vi "detect modules.vi"(8 "error in":errorcluster, 10 "C Series module in":refnum<class "C Series Module.lvclass">, 11 "chassis in":refnum<class "Chassis.lvclass">) -> (0 "error out":errorcluster, 2 "C Series module out":refnum<class "C Series Module.lvclass">, 3 "chassis out":refnum<class "Chassis.lvclass">)   [LabVIEW 2014, in "SMI.lvlib" / "C Series Module.lvclass"]
uses:
  C Series Module.lvclass
  Chassis/Chassis.lvclass
  <vilib>/FPGAPlugInAG/Dynamic/niLvFpga_Close_Dynamic.vi
  <vilib>/FPGAPlugInAG/Dynamic/niLvFpga_Run_Dynamic.vi
  <vilib>/FPGAPlugInAG/Dynamic/niLvFpga_Reset_Dynamic.vi
  Device/read device class.vi
  Device/read product name.vi
  <vilib>/regexp/Match Regular Expression.xnode
  <vilib>/rvi/interface/nirviCloseFPGA/nirviCloseFPGA.xnode
  <vilib>/rvi/interface/nirviMethod/nirviMethod.xnode
  Module/Module.lvclass
  SMI.lvlib
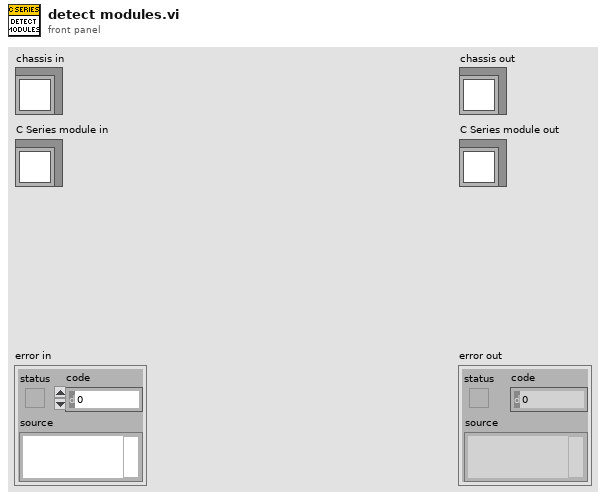
[diagram p1: front panel]
types:
  T1 = typedef "SMI.lvlib/Module.lvclass/module information.ctl" = cluster{"vendor name":string, "product name":string, "product ID":u16, "serial number":string}
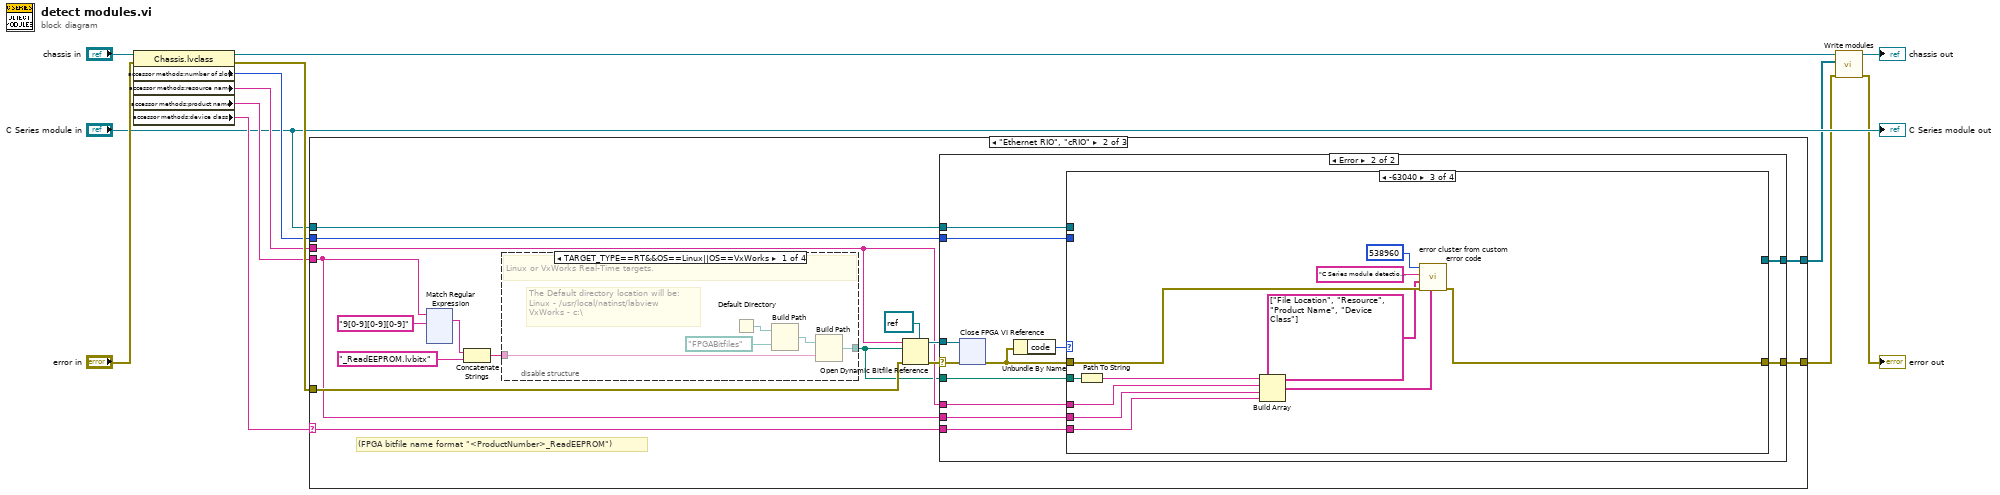
[diagram p0: block diagram]
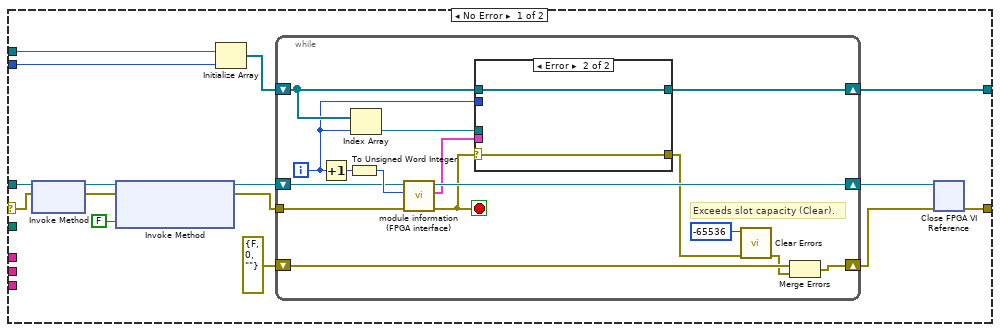
[diagram p3: hidden frame]
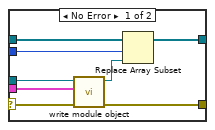
[diagram p4: hidden frame]
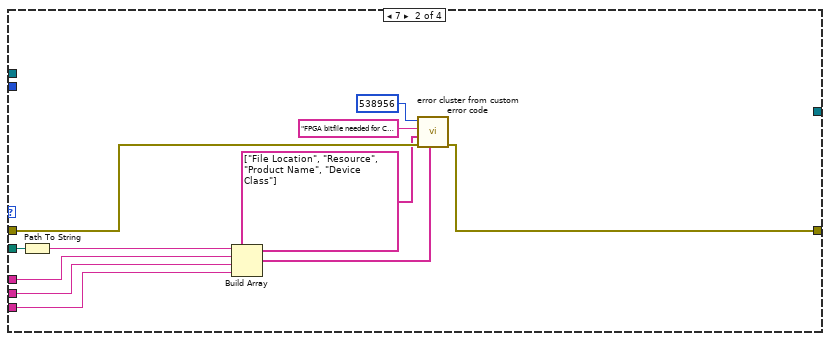
[diagram p6: hidden frame]
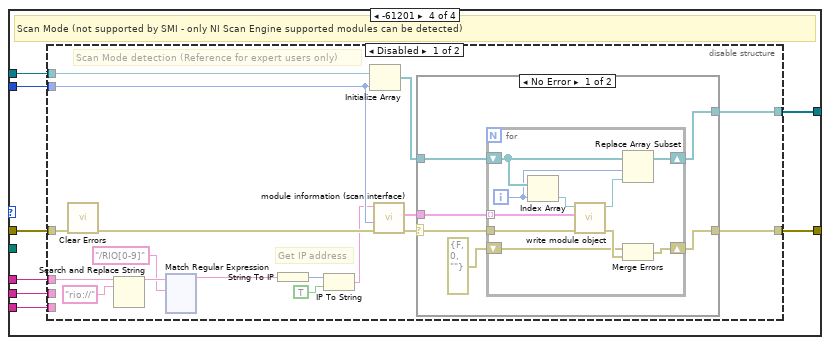
[diagram p7: hidden frame]
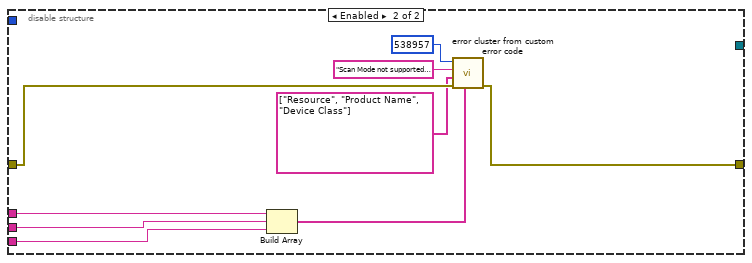
[diagram p9: hidden frame]
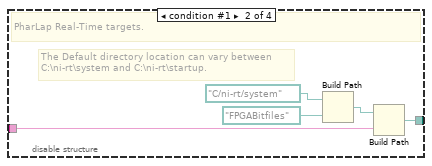
[diagram p10: hidden frame]
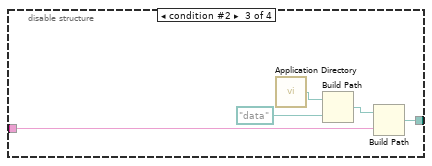
[diagram p11: hidden frame]
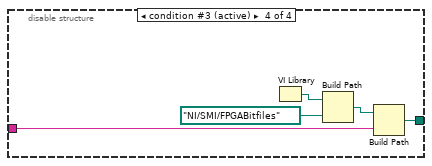
[diagram p12: hidden frame]
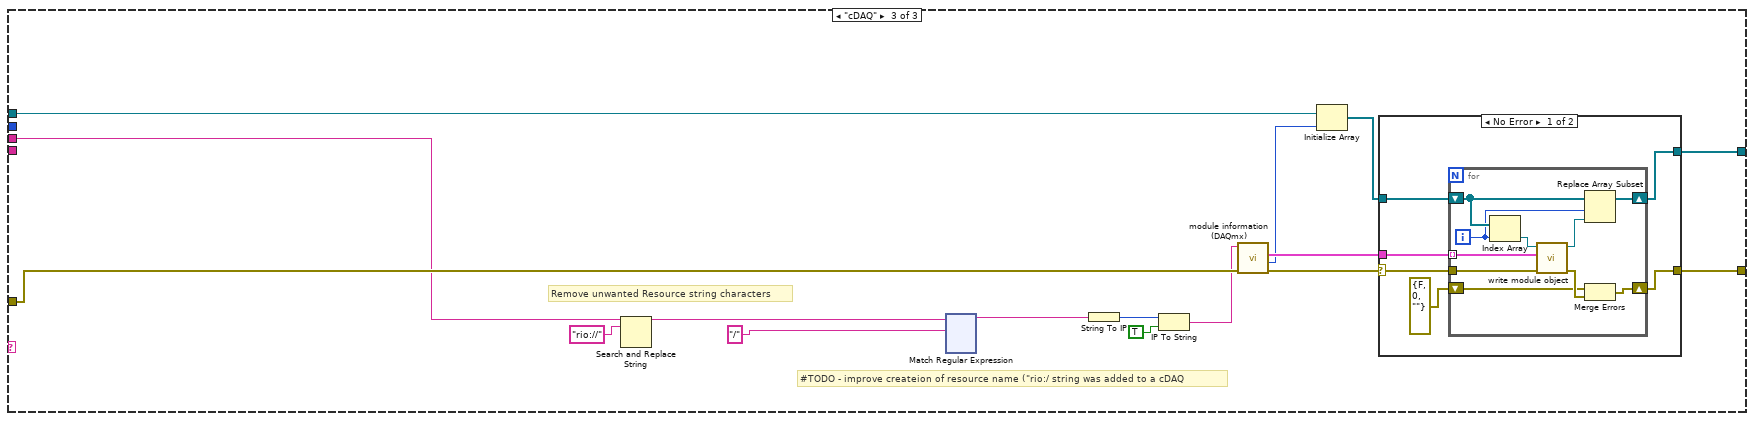
[diagram p13: hidden frame]
diagram:
  n1 = property class="Chassis.lvclass"(reference="chassis in", error in="error in") -> (reference out=w6:refnum<class "Chassis.lvclass">, error out=w12:errorcluster, "accessor methods:number of slots"=w7:i32, "accessor methods:resource name"=w8:string, "accessor methods:product name"=w9:string, "accessor methods:device class"=w10:string)
  n2 = case shown="\"Ethernet RIO\", \"cRIO\"" w10 {
    selector: w10 -> [_ w15 _]
    tunnel: [w14 w19 w418] -> w2
    tunnel: w12 -> [w14 w26 w421]
    tunnel: w9 -> [_ w16 _]
    tunnel: w8 -> [_ w18 w417]
    tunnel: w7 -> [_ w22 _]
    tunnel: "C Series module in" -> [_ w23 w420]
    tunnel: [_ w20 w419] -> w3
    frame Default {
      # "#TODO - Re-create block diagram (from lv2016 reference)."
    }
    frame "Ethernet RIO", "cRIO" {
      # "(FPGA bitfile name format \"<ProductNumber>_ReadEEPROM\")"
      n3 = xnode "Match Regular Expression"("input string"=w16, "regular expression"="9[0-9][0-9][0-9]") -> ("whole match"=w29:string)  [unwired: 4 in, 4 out]
      n4 = Concatenate Strings(w29, "_ReadEEPROM.lvbitx" ("string")) -> (w27:string)
      n5 = disable-structure shown="TARGET_TYPE==RT&&OS==Linux||OS==VxWorks" {
        disable-tunnel: w27 -> [w273 w279 w284 w288]
        disable-tunnel: [w272 w278 w283 w287] -> w17
        frame condition #0 {
          # "The Default directory location will be:\nLinux - /usr/local/natinst/labview\nVxWorks - c:\\"
          # "Linux or VxWorks Real-Time targets."
          n6 = Default Directory() -> (w276:path)
          n7 = Build Path(base path=w276, name or relative path=path "FPGABitfiles") -> (appended path=w274:path)
          n8 = Build Path(base path=w274, name or relative path=w273) -> (appended path=w272:path)
        }
        frame condition #1 {
          # "The Default directory location can vary between\nC:\\ni-rt\\system and C:\\ni-rt\\startup."
          # "PharLap Real-Time targets."
          n9 = Build Path(base path=path "C:/ni-rt/system", name or relative path=path "FPGABitfiles") -> (appended path=w280:path)
          n10 = Build Path(base path=w280, name or relative path=w279) -> (appended path=w278:path)
        }
        frame condition #2 {
          n11 = call <vilib>:"Application Directory.vi"() -> ("Application Directory"=w282:path)
          n12 = Build Path(base path=w282, name or relative path=path "data") -> (appended path=w285:path)
          n13 = Build Path(base path=w285, name or relative path=w284) -> (appended path=w283:path)
        }
        frame condition #3 (active) {
          n14 = VI Library() -> (path=w291:path)
          n15 = Build Path(base path=w291, name or relative path=path "NI/SMI/FPGABitfiles") -> (appended path=w289:path)
          n16 = Build Path(base path=w289, name or relative path=w288) -> (appended path=w287:path)
        }
      }
      n17 = Open Dynamic Bitfile Reference(0:w18, 1:w17, 3:w26, 4:refnum<k20> refnum ("Refnum in")) -> (5:w24:refnum<k20>, 8:w25:errorcluster)  [unwired: 1 in]
      n18 = case shown="Error" w25 {
        selector: w25 -> [w36 w75]
        tunnel: w24 -> [w37 w76]
        tunnel: w23 -> [w45 w82]
        tunnel: w22 -> [w44 w81]
        tunnel: [w42 w79] -> w20
        tunnel: [w38 w78] -> w19
        tunnel: w18 -> [_ w80]
        tunnel: w17 -> [_ w77]
        tunnel: w16 -> [_ w72]
        tunnel: w15 -> [_ w73]
        frame No Error {
          n19 = xnode "Invoke Method"("FPGA VI Reference In"=w37, "error in"=w36) -> ("FPGA VI Reference Out"=w35:refnum<k20>, "error out"=w34:errorcluster)
          n20 = xnode "Invoke Method"("FPGA VI Reference In"=w35, "error in"=w34, "Wait Until Done (F)"=FALSE) -> ("FPGA VI Reference Out"=w33:refnum<k20>, "error out"=w32:errorcluster)
          n21 = Initialize Array(w45, w44) -> (w43:refnum<class "C Series Module.lvclass">[])
          n22 = while {
            shift-right: [w53] -> w42
            shift-left: w43 -> [w54]
            tunnel: w32 -> [w61]
            shift-right: [w57] -> w40
            shift-left: w33 -> [w58]
            shift-right: [w48] -> w39
            shift-left: errorcluster {"status"=FALSE, "code"=0, "source"=""} ("error constant") -> [w49]
            i -> [w52]
            stop <- w51 stop-if-true
            # "Exceeds slot capacity (Clear)."
            n23 = Increment(x=w52) -> (x+1=w60:i32)
            n24 = To Unsigned Word Integer(number=w60) -> (unsigned 16bit integer=w59:u16)
            n25 = Index Array(array=w54, index=w52) -> (element=w56:refnum<class "C Series Module.lvclass">)
            n26 = call "module information (FPGA interface).vi"("error in"=w61, "Module"=w59, "Refnum in"=w58) -> ("error out"=w51:errorcluster, "Module Information"=w55:T1, "Refnum out"=w57:refnum<k20>)  [unwired: 6 in]
            n27 = case shown="Error" w51 {
              selector: w51 -> [w68 w70]
              tunnel: w56 -> [w69 _]
              tunnel: w55 -> [w67 _]
              tunnel: w54 -> [w66 w71]
              tunnel: [w65 w71] -> w53
              tunnel: w52 -> [w63 _]
              tunnel: [w62 w70] -> w50
              frame No Error {
                n28 = call "write module object.vi"("error in"=w68, "module information"=w67, "Module in"=w69) -> ("error out"=w62:errorcluster, "Module out"=w64:refnum<class "C Series Module.lvclass">)  [unwired: 7 in]
                n29 = Replace Array Subset(array=w66, new element=w64, index=w63) -> (w65:refnum<class "C Series Module.lvclass">[])
              }
              frame Error {
              }
            }
            n30 = call <vilib>:"Clear Errors.vi"("error in (no error)"=w50, "specific error code to clear (0: all)"=-65536) -> ("error out"=w47:errorcluster)  [unwired: 4 in, 1 out]
            n31 = Merge Errors(w49, w47) -> (w48:errorcluster)
          }
          n32 = xnode "Close FPGA VI Reference"("FPGA VI Reference In"=w40, "error in"=w39) -> ("error out"=w38:errorcluster)
        }
        frame Error {
          n33 = xnode "Close FPGA VI Reference"("FPGA VI Reference In"=w76, "error in"=w75) -> ("error out"=w74:errorcluster)
          n34 = Unbundle By Name(w74) -> ("code"=w83:i32)
          n35 = case shown="-63040" w83 {
            tunnel: w74 -> [w84 w92 w103 w114]
            tunnel: w82 -> [_ _ _ w113]
            tunnel: w81 -> [_ _ _ w112]
            tunnel: w80 -> [_ w91 w102 w111]
            tunnel: [_ _ _ w110] -> w79
            tunnel: [w84 w94 w105 w109] -> w78
            tunnel: w77 -> [_ w95 w106 _]
            tunnel: w73 -> [_ w89 w100 w107]
            tunnel: w72 -> [_ w90 w101 w108]
            frame Default {
            }
            frame 7 {
              n36 = Path To String(path=w95) -> (string=w93:string)
              n37 = Build Array(w93, w91, w90, w89) -> (w87:string[])
              n38 = call "error cluster from custom error code.vi"("string values"=w87, "error in"=w92, "keys"=string[] ["File Location", "Resource", "Product Name", "Device Class"], "error message"="FPGA bitfile needed for C Series module detection was not found in the expected file location.", "custom error code (0)"=538956 ("error code (0)")) -> ("error out"=w94:errorcluster)  [unwired: 6 in]
            }
            frame -63040 {
              n39 = Path To String(path=w106) -> (string=w104:string)
              n40 = Build Array(w104, w102, w101, w100) -> (w98:string[])
              n41 = call "error cluster from custom error code.vi"("string values"=w98, "error in"=w103, "keys"=string[] ["File Location", "Resource", "Product Name", "Device Class"], "error message"="C Series module detection is not supported for remote chassis connected to a secondary network adapter.", "custom error code (0)"=538960 ("error code (0)")) -> ("error out"=w105:errorcluster)  [unwired: 6 in]
            }
            frame -61201 {
              # "Scan Mode (not supported by SMI - only NI Scan Engine supported modules can be detected)"
              n42 = disable-structure shown="Disabled" {
                disable-tunnel: w114 -> [w131 w268]
                disable-tunnel: w113 -> [w130 _]
                disable-tunnel: w112 -> [w129 _]
                disable-tunnel: w111 -> [w125 w271]
                disable-tunnel: [w120 _] -> w110
                disable-tunnel: [w119 w267] -> w109
                disable-tunnel: w108 -> [_ w270]
                disable-tunnel: w107 -> [_ w269]
                frame Disabled {
                  # "Get IP address"
                  # "Scan Mode detection (Reference for expert users only)"
                  n43 = call <vilib>:"Clear Errors.vi"("error in (no error)"=w131) -> ("error out"=w126:errorcluster)  [unwired: 5 in, 1 out]
                  n44 = Search and Replace String(input string=w125, search string="rio://") -> (result string=w123:string)  [unwired: 6 in, 3 out]
                  n45 = xnode "Match Regular Expression"("input string"=w123, "regular expression"="/RIO[0-9]") -> ("before match"=w116:string)  [unwired: 4 in, 4 out]
                  n46 = String To IP(1:w116) -> (0:w118:u32)
                  n47 = IP To String(1:TRUE ("dot notation? (F)"), 2:w118) -> (0:w115:string)
                  n48 = Initialize Array(w130, w129) -> (w121:refnum<class "C Series Module.lvclass">[])
                  n49 = call "module information (scan interface).vi"("error in"=w126, "number of slots"=w129, "IP address (localhost)"=w115) -> ("error out"=w128:errorcluster, "module information"=w127:T1[])  [unwired: 7 in]
                  n50 = case shown="No Error" w128 {
                    selector: w128 -> [w248 w262]
                    tunnel: w127 -> [w251 _]
                    tunnel: w121 -> [w250 _]
                    tunnel: [w247 _] -> w120
                    tunnel: [w246 w262] -> w119
                    frame No Error {
                      n51 = for {
                        tunnel: w251 -> [w261] mode=indexing
                        shift-right: [w254] -> w247
                        shift-left: w250 -> [w255]
                        shift-right: [w256] -> w246
                        shift-left: errorcluster {"status"=FALSE, "code"=0, "source"=""} ("error constant") -> [w258]
                        tunnel: w248 -> [w260]
                        i -> [w253]
                        n52 = Index Array(array=w255, index=w253) -> (element=w257:refnum<class "C Series Module.lvclass">)
                        n53 = call "write module object.vi"("error in"=w260, "module information"=w261, "Module in"=w257) -> ("error out"=w259:errorcluster, "Module out"=w252:refnum<class "C Series Module.lvclass">)  [unwired: 7 in]
                        n54 = Replace Array Subset(array=w255, new element=w252, index=w253) -> (w254:refnum<class "C Series Module.lvclass">[])
                        n55 = Merge Errors(w258, w259) -> (w256:errorcluster)
                      }
                    }
                    frame Error {
                    }
                  }
                }
                frame Enabled {
                  n56 = Build Array(w271, w270, w269) -> (w265:string[])
                  n57 = call "error cluster from custom error code.vi"("string values"=w265, "error in"=w268, "keys"=string[] ["Resource", "Product Name", "Device Class"], "error message"="Scan Mode not supported for C Series module detection.", "custom error code (0)"=538957 ("error code (0)")) -> ("error out"=w267:errorcluster)  [unwired: 6 in]
                }
              }
            }
          }
        }
      }
    }
    frame "cDAQ" {
      # "#TODO - improve createion of resource name (\"rio:/ string was added to a cDAQ"
      # "Remove unwanted Resource string characters"
      n58 = Search and Replace String(input string=w417, search string="rio://") -> (result string=w413:string)  [unwired: 6 in, 3 out]
      n59 = xnode "Match Regular Expression"("input string"=w413, "regular expression"="/") -> ("before match"=w409:string)  [unwired: 4 in, 4 out]
      n60 = String To IP(1:w409) -> (0:w408:u32)
      n61 = IP To String(1:TRUE ("dot notation? (F)"), 2:w408) -> (0:w406:string)
      n62 = call "module information (DAQmx).vi"("error in"=w421, "IP address (localhost)"=w406) -> ("error out"=w416:errorcluster, "number of slots"=w410:i32, "module information"=w415:T1[])  [unwired: 7 in]
      n63 = Initialize Array(w420, w410) -> (w411:refnum<class "C Series Module.lvclass">[])
      n64 = case shown="No Error" w416 {
        selector: w416 -> [w538 w552]
        tunnel: w415 -> [w541 _]
        tunnel: w411 -> [w540 _]
        tunnel: [w537 _] -> w419
        tunnel: [w536 w552] -> w418
        frame No Error {
          n65 = for {
            tunnel: w541 -> [w551] mode=indexing
            shift-right: [w544] -> w537
            shift-left: w540 -> [w545]
            shift-right: [w546] -> w536
            shift-left: errorcluster {"status"=FALSE, "code"=0, "source"=""} ("error constant") -> [w548]
            tunnel: w538 -> [w550]
            i -> [w543]
            n66 = Index Array(array=w545, index=w543) -> (element=w547:refnum<class "C Series Module.lvclass">)
            n67 = call "write module object.vi"("error in"=w550, "module information"=w551, "Module in"=w547) -> ("error out"=w549:errorcluster, "Module out"=w542:refnum<class "C Series Module.lvclass">)  [unwired: 7 in]
            n68 = Replace Array Subset(array=w545, new element=w542, index=w543) -> (w544:refnum<class "C Series Module.lvclass">[])
            n69 = Merge Errors(w548, w549) -> (w546:errorcluster)
          }
        }
        frame Error {
        }
      }
    }
  }
  n70 = call-dynamic "Write modules.vi"("error in (no error)"=w2, "modules"=w3, "Chassis in"=w6) -> ("error out"=→"error out":errorcluster, "Chassis out"=→"chassis out":refnum<class "Chassis.lvclass">)  [unwired: 7 in]
  "C Series module out" <- "C Series module in"
